vi "Line Configuration Dialog.vi"(8 "error in":errorcluster, 9 "engine configuration in":refnum<class "engine configuration.lvclass">, 10 "tag bus configurable plugin module configuration":refnum<class "J1939 configuration.lvclass">, 11 "Line":T4={"channel"=refnum, "XNET Signal"="CANEventSignal1\nNIXNET_example.CAN_Cluster"}) -> (0 "error out":errorcluster, 1 "success":bool, 2 "changed":bool, 3 "Mappings out":T3={"Line"={"channel"=refnum, "XNET Signal"="CANEventSignal1\nNIXNET_example.CAN_Cluster"}, "Maps"=[]})   [LabVIEW 2015, in "J1939 editor node.lvclass"]
doc: "A dialog for allowing a user to specify the values of a new line."
uses:
  J1939 editor node.lvclass
  module/configuration/Line.ctl
  <vilib>/NI/Tag Bus Module Framework/channel/TBM channel.lvclass
  Mappings.ctl
  Map.ctl
  permissions.ctl
  <vilib>/NI/Module Execution Interface/Engine Configuration/engine configuration.lvclass
  module/configuration/J1939 configuration.lvclass
  <vilib>/NI/Tag Bus/tag/Data Type.ctl
  <vilib>/NI/Tag Bus Module Framework/channel/TBM channel.lvclass/TBM channel.ctl
  <vilib>/NI/Configuration Framework/serializable configuration/NISE_CEF_serializable configuration.lvclass/NISE_CEF_serializable configuration.ctl
  <vilib>/NI/Tag Bus/tag/tag descriptor.lvclass/tag descriptor.ctl
  <vilib>/NI/Tag Bus Module Framework/channel/channel classification.ctl
  <vilib>/NI/Tag Bus/tag/write tag name.vi
  <vilib>/NI/Tag Bus/tag/write data type.vi
  <vilib>/NI/Tag Bus Module Framework/channel/Write channel classification.vi
  <vilib>/NI/Configuration Framework/serializable configuration/Read UID.vi
  <vilib>/NI/Tag Bus Module Framework/channel/Read channel classification.vi
  <vilib>/Utility/LVClass/Get LV Class Name.vi
  <vilib>/NI/Configuration Framework/error generator/NISE_error generator.vi
  <vilib>/NI/Tag Bus/tag/tag descriptor.lvclass
  <vilib>/NI/DCAF UI Toolkit/Controls/DCAF UI Elements.lvlib
panel:
  out "Data Type":T1
  in  "XNET Signal":refnum<k21>="CANEventSignal1\nNIXNET_example.CAN_Cluster"
  out "errors":string
  in  "Access Type":T2
  in  "Available Tags":i32(listbox)
  in  "cancel":bool
  in  "ok":bool
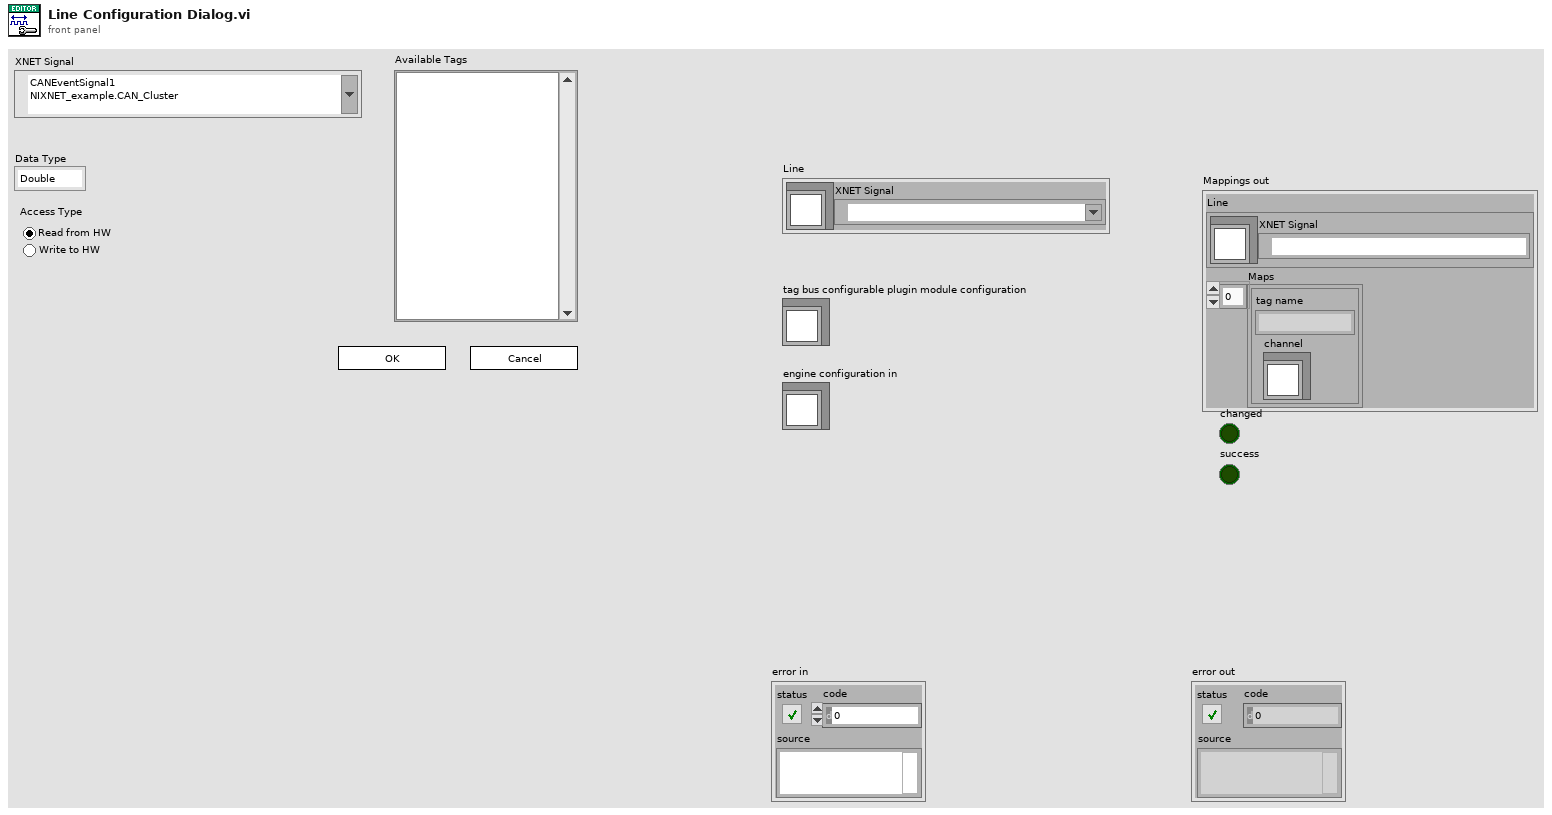
[diagram p1: front panel]
types:
  T1 = typedef "tag bus.lvlib/tag descriptor.lvclass/Data Type.ctl" = enum16{"Double", "Single", "I64", "I32", "I16", "I8", "U64", "U32", "U16", "U8", "Boolean", "String", "Array of Double", "Array of Single", "Array of I64", "Array of I32", "Array of I16", "Array of I8", "Array of U64", "Array of U32", "Array of U16", "Array of U8", "Array of Boolean", "Array of String"}
  T2 = typedef "J1939 editor node.lvclass/permissions.ctl" = enum32{"Read from HW", "Write to HW"}
  T3 = typedef "J1939 editor node.lvclass/Mappings.ctl" = cluster{"Line":T4, "Maps":T5[]}
  T4 = typedef "J1939 configuration.lvclass/Line.ctl" = cluster{"channel":refnum<class "TBM channel.lvclass">, "XNET Signal":refnum<k21>}
  T5 = typedef "J1939 editor node.lvclass/Map.ctl" = cluster{"channel":refnum<class "TBM channel.lvclass">, "tag name":string}
  T6 = typedef "TBM channel.lvclass/channel classification.ctl" = enum16{"input data", "output data", "processing parameter", "processing result"}
  T7 = enum8{"Enabled", "Disabled", "Disabled and Grayed Out"}
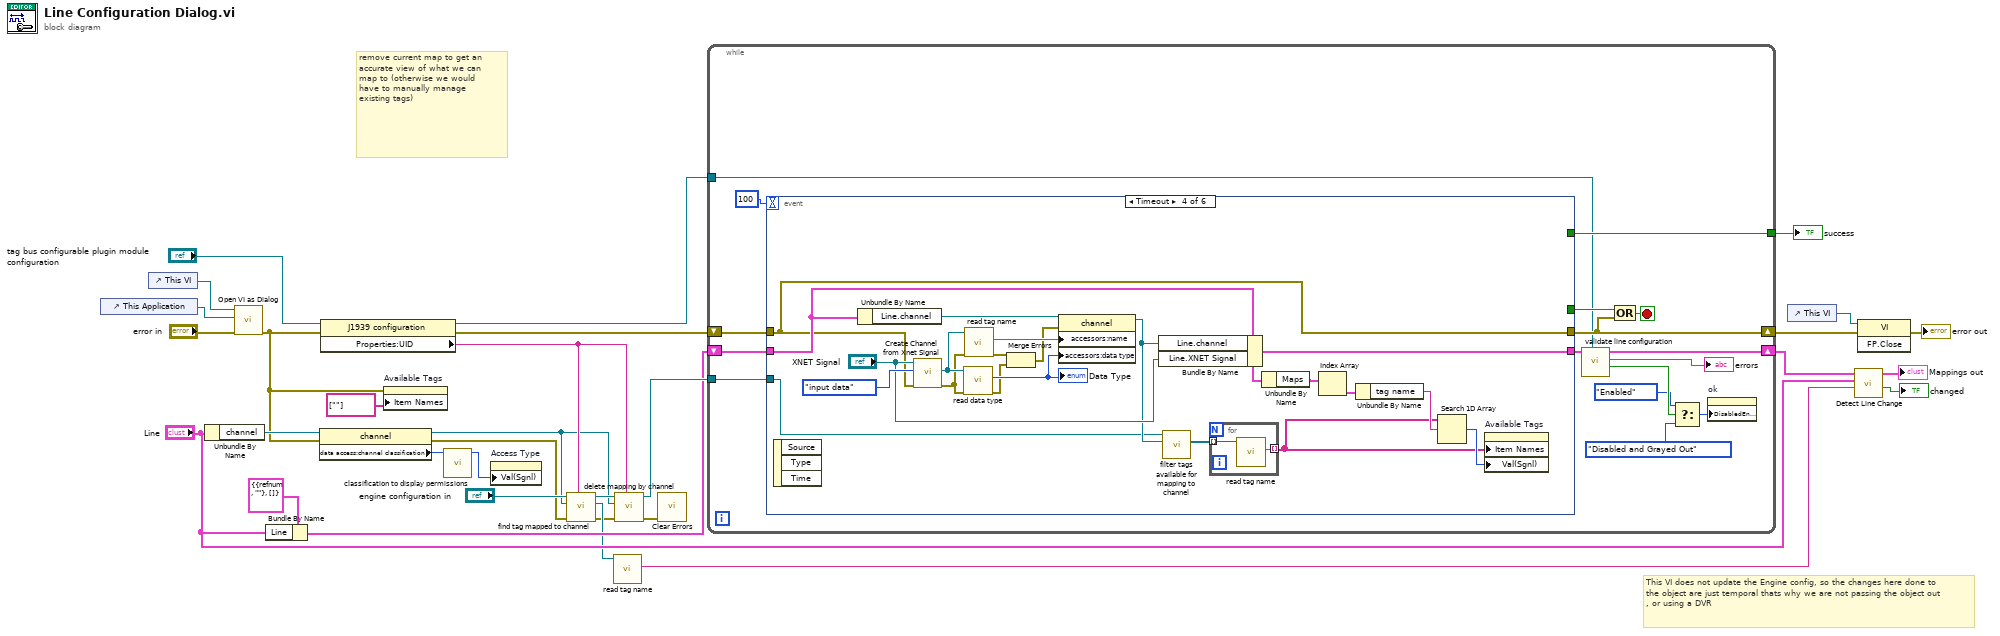
[diagram p0: block diagram]
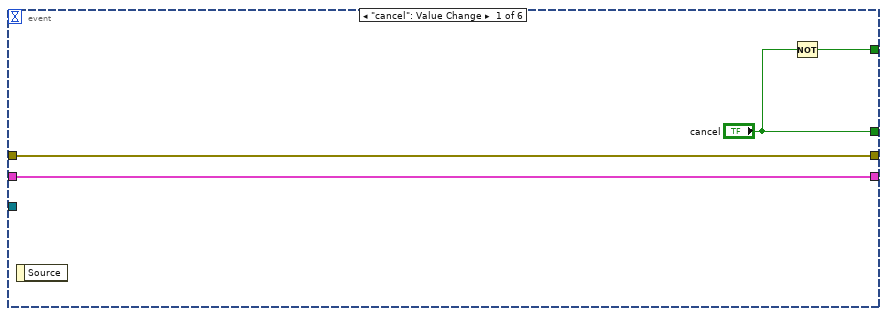
[diagram p2: hidden frame]
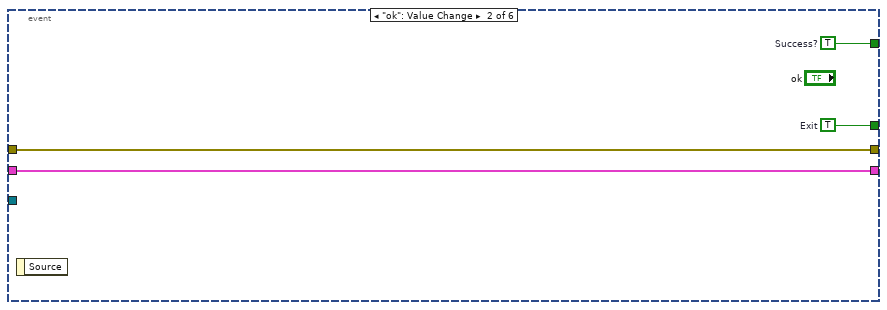
[diagram p3: hidden frame]
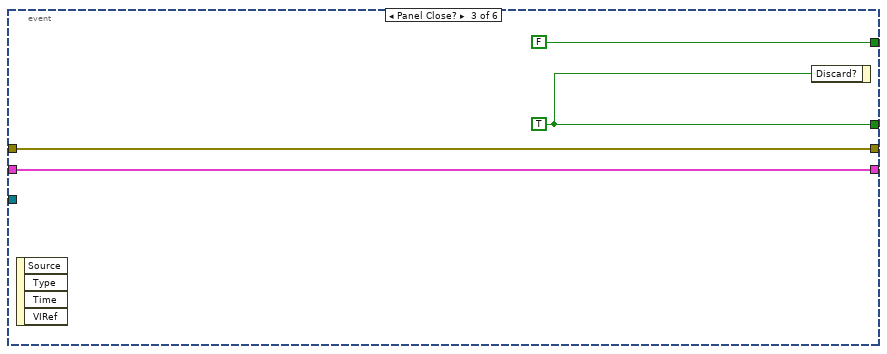
[diagram p4: hidden frame]
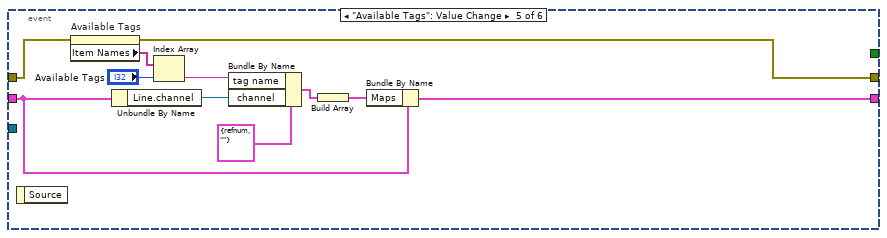
[diagram p5: hidden frame]
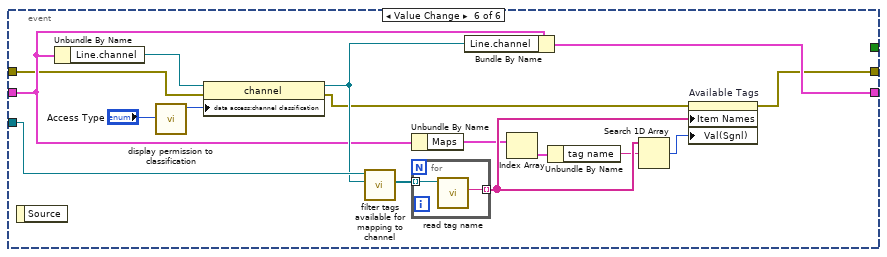
[diagram p6: hidden frame]
diagram:
  # "This VI does not update the Engine config, so the changes here done to the object are just temporal thats why we are not passing the object out , or using a DVR"
  # "remove current map to get an accurate view of what we can map to (otherwise we would have to manually manage existing tags)"
  n1 = control-ref of="This Application"() -> (w16:refnum<vi>)
  n2 = control-ref of="This VI"() -> (w17:refnum<vi>)
  n3 = Unbundle By Name("Line") -> ("channel"=w27:refnum<class "TBM channel.lvclass">)
  n4 = call <vilib>:"Open VI as Dialog.vi"("error in (no error)"="error in", "This Application"=w16, "VI in"=w17) -> ("error out"=w14:errorcluster)  [unwired: 8 in]
  n5 = Bundle By Name(cluster=T3 {"Line"={"channel"=refnum, "XNET Signal"=""}, "Maps"=[]} ("Mappings out"), "Line"="Line") -> (w19:T3)
  n6 = property class="channel"(reference=w27, error in=w14) -> (reference out=w10:refnum<class "TBM channel.lvclass">, error out=w7:errorcluster, "data access:channel classification"=w28:T6)
  n7 = property class="J1939 configuration"(reference="tag bus configurable plugin module configuration", error in=w14) -> (reference out=w29:refnum<class "J1939 configuration.lvclass">, error out=w22:errorcluster, "Properties:UID"=w12:string)
  n8 = property on="Available Tags" class="LstBox (strict)"(error in=w14, "Item Names"=string[] [""]) -> ()  [unwired: 1 in, 2 out]
  n9 = call "classification to display permissions.vi"("channel classification"=w28) -> ("permissions"=w25:T2)  [unwired: 10 in]
  n10 = property on="Access Type" class="RadioBtnsControl (strict)"("Val(Sgnl)"=w25) -> ()  [unwired: 2 in, 2 out]
  n11 = call <vilib>:"find tag mapped to channel.vi"("owner"=w12, "error in"=w7, "channel"=w10, "engine configuration in"="engine configuration in") -> ("error out"=w6:errorcluster, "tag"=w9:refnum<class "tag descriptor.lvclass">, "engine configuration out"=w11:refnum<class "engine configuration.lvclass">)  [unwired: 5 in]
  n12 = call <vilib>:"read tag name.vi"("system tag in"=w9) -> ("name"=w8:string)  [unwired: 8 in, 2 out]
  n13 = call <vilib>:"delete mapping by channel.vi"("owner ID"=w12, "error in"=w6, "channel"=w10, "engine configuration in"=w11) -> ("error out"=w24:errorcluster, "engine configuration out"=w30:refnum<class "engine configuration.lvclass">)  [unwired: 6 in]
  n14 = call <vilib>:"Clear Errors.vi"("error in (no error)"=w24) -> ()  [unwired: 5 in, 2 out]
  n15 = while {
    shift-right: [w39] -> w2
    shift-left: w22 -> [w46]
    tunnel: [w45] -> w31
    shift-right: [w40] -> w18
    shift-left: w19 -> [w42]
    tunnel: w30 -> [w47]
    tunnel: w29 -> [w34]
    stop <- w43 stop-if-true
    n16 = event shown="[3] Timeout" {
      selector: _ -> [_ _ _ _ _ _]
      dyn-events: _ -> [_ _ _ _ _ _]
      timeout: 100 -> [_ _ _ _ _ _]
      tunnel: w47 -> [_ _ _ w67 _ w107]
      tunnel: w46 -> [w51 w55 w59 w64 w84 w101]
      tunnel: [w51 w55 w59 w64 w83 w99] -> w39
      tunnel: [w50 w52 FALSE _ _ _] -> w45
      tunnel: ["cancel" w53 w57 _ _ _] -> w44
      tunnel: w42 -> [w48 w54 w56 w70 w88 w105]
      tunnel: [w48 w54 w56 w80 w85 w104] -> w41
      event "cancel": Value Change {
        n17 = event-data() -> ()  [unwired: 1 in, 1 out]
        n18 = Not(x="cancel") -> (.not. x?=w50:bool)
      }
      event "ok": Value Change {
        w52 = TRUE  # Success?
        w53 = TRUE  # Exit
        n19 = event-data() -> ()  [unwired: 1 in, 1 out]
      }
      event Panel Close? {
        w57 = TRUE ("cancel")
        n20 = event-data() -> ()  [unwired: 1 in, 4 out]
        n21 = event-data("Discard?"=w57) -> ()  [unwired: 1 in, 1 out]
      }
      event Timeout {
        n22 = event-data() -> ()  [unwired: 1 in, 3 out]
        n23 = Unbundle By Name(w70) -> ("Line.channel"=w79:refnum<class "TBM channel.lvclass">)
        n24 = call "Create Channel from Xnet Signal.vi"("error in (no error)"=w64, "channel classification"=channel_classification."input data", "XNET Signal"="XNET Signal") -> ("error out"=w63:errorcluster, "channel"=w77:refnum<class "TBM channel.lvclass">)  [unwired: 6 in, 1 out]
        n25 = call <vilib>:"read data type.vi"("error in"=w63, "system tag in"=w77) -> ("error out"=w60:errorcluster, "data type"=w75:T1)  [unwired: 7 in, 1 out]
        "Data Type" <- w75
        n26 = call <vilib>:"read tag name.vi"("error in"=w63, "system tag in"=w77) -> ("error out"=w62:errorcluster, "name"=w76:string)  [unwired: 7 in, 1 out]
        n27 = Merge Errors(w62, w60) -> (w61:errorcluster)
        n28 = property class="channel"(reference=w79, error in=w61, "accessors:name"=w76, "accessors:data type"=w75) -> (reference out=w68:refnum<class "TBM channel.lvclass">)  [unwired: 1 out]
        n29 = Bundle By Name(cluster=w70, "Line.channel"=w68, "Line.XNET Signal"="XNET Signal") -> (w80:T3)
        n30 = call-dynamic "filter tags available for mapping to channel.vi"("channel to map to"=w68, "engine configuration in"=w67) -> ("filtered tags"=w69:refnum<class "tag descriptor.lvclass">[])  [unwired: 8 in, 1 out]
        n31 = for {
          tunnel: w69 -> [w82] mode=indexing
          tunnel: [w81] -> w65 mode=indexing
          n32 = call <vilib>:"read tag name.vi"("system tag in"=w82) -> ("name"=w81:string)  [unwired: 8 in, 2 out]
        }
        n33 = Unbundle By Name(w70) -> ("Maps"=w73:T5[])
        n34 = Index Array(array=w73) -> (element=w72:T5)  [unwired: 1 in]
        n35 = Unbundle By Name(w72) -> ("tag name"=w71:string)
        n36 = Search 1D Array(1D array=w65, element=w71) -> (index of element=w66:i32)  [unwired: 1 in]
        n37 = property on="Available Tags" class="LstBox (strict)"("Item Names"=w65, "Val(Sgnl)"=w66) -> ()  [unwired: 2 in, 2 out]
      }
      event "Available Tags": Value Change {
        n38 = event-data() -> ()  [unwired: 1 in, 1 out]
        n39 = property on="Available Tags" class="LstBox (strict)"(error in=w84) -> (error out=w83:errorcluster, "Item Names"=w92:string[])  [unwired: 1 in, 1 out]
        n40 = Unbundle By Name(w88) -> ("Line.channel"=w89:refnum<class "TBM channel.lvclass">)
        n41 = Index Array(array=w92, index="Available Tags") -> (element=w91:string)
        n42 = Bundle By Name(cluster=T5 {"channel"=refnum, "tag name"=""} ("Map"), "tag name"=w91, "channel"=w89) -> (w87:T5)
        n43 = Build Array(w87) -> (w86:T5[])
        n44 = Bundle By Name(cluster=w88, "Maps"=w86) -> (w85:T3)
      }
      event Value Change {
        n45 = event-data() -> ()  [unwired: 1 in, 1 out]
        n46 = Unbundle By Name(w105) -> ("Line.channel"=w109:refnum<class "TBM channel.lvclass">)
        n47 = call "display permission to classification.vi"("display permissions"="Access Type") -> ("channel classification"=w108:T6)  [unwired: 10 in]
        n48 = property class="channel"(reference=w109, error in=w101, "data access:channel classification"=w108) -> (reference out=w106:refnum<class "TBM channel.lvclass">, error out=w100:errorcluster)
        n49 = call-dynamic "filter tags available for mapping to channel.vi"("channel to map to"=w106, "engine configuration in"=w107) -> ("filtered tags"=w103:refnum<class "tag descriptor.lvclass">[])  [unwired: 8 in, 1 out]
        n50 = Unbundle By Name(w105) -> ("Maps"=w96:T5[])
        n51 = for {
          tunnel: w103 -> [w111] mode=indexing
          tunnel: [w110] -> w98 mode=indexing
          n52 = call <vilib>:"read tag name.vi"("system tag in"=w111) -> ("name"=w110:string)  [unwired: 8 in, 2 out]
        }
        n53 = Bundle By Name(cluster=w105, "Line.channel"=w106) -> (w104:T3)
        n54 = Index Array(array=w96) -> (element=w95:T5)  [unwired: 1 in]
        n55 = Unbundle By Name(w95) -> ("tag name"=w94:string)
        n56 = Search 1D Array(1D array=w98, element=w94) -> (index of element=w97:i32)  [unwired: 1 in]
        n57 = property on="Available Tags" class="LstBox (strict)"(error in=w100, "Item Names"=w98, "Val(Sgnl)"=w97) -> (error out=w99:errorcluster)  [unwired: 1 in, 1 out]
      }
    }
    n58 = call "validate line configuration.vi"("Module Config"=w34, "Mappings in"=w41) -> ("valid?"=w38:bool, "errors"=→"errors":string, "Mappings out"=w40:T3)  [unwired: 7 in]
    n59 = Compound Arithmetic op=OR(w44, w39) -> (w43:bool)
    n60 = Select(t=T7."Enabled" ("Disabled"), s=w38, f=T7."Disabled and Grayed Out") -> (s? t:f=w35:T7)
    n61 = property on="ok" class="Bool"("DisabledEnum"=w35) -> ()  [unwired: 2 in, 2 out]
  }
  "success" <- w31
  n62 = control-ref of="This VI"() -> (w3:refnum<vi>)
  n63 = call "Detect Line Change.vi"("Origianl Tag"=w8, "Original Line"="Line", "Final Mappings in"=w18) -> ("Boolean"=→"changed":bool, "Final Mappings out"=→"Mappings out":T3)  [unwired: 7 in]
  n64 = invoke class="VI" method="FP.Close"(reference=w3, error in=w2) -> (error out=→"error out":errorcluster)  [unwired: 1 in, 2 out]
